vi "电缸控制.vi"(1 "步序号":u32, 2 "枚举":enum16{"开机", "返回原点", "定位运转", "报警复位"}(ring), 3 "输出设备":tag) -> (0 "error out":errorcluster caption="错误输出")   [LabVIEW 2014]
uses:
  <vilib>/DAQmx/create/channels.llb/DAQmx Create Channel (DO-Digital Output).vi
  <vilib>/DAQmx/write.llb/DAQmx Write (Digital 1D Bool 1Chan 1Samp).vi
panel:
  in  "步信息":T1
  in  "人工输出":T2
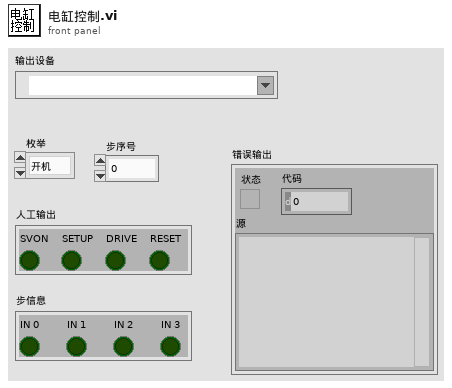
[diagram p1: front panel]
types:
  T1 = cluster{"IN 0":bool, "IN 1":bool, "IN 2":bool, "IN 3":bool}
  T2 = cluster{"SVON":bool, "SETUP":bool, "DRIVE":bool, "RESET":bool}
  T3 = cluster{"Boolean array[0]":bool, "Boolean array[1]":bool, "Boolean array[2]":bool, "Boolean array[3]":bool}
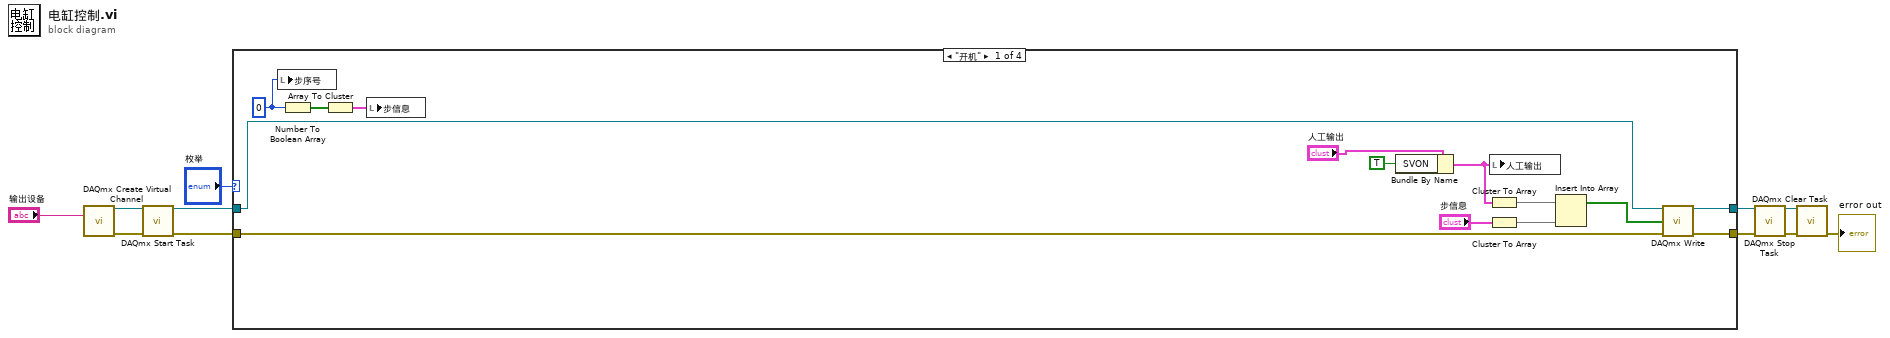
[diagram p0: block diagram]
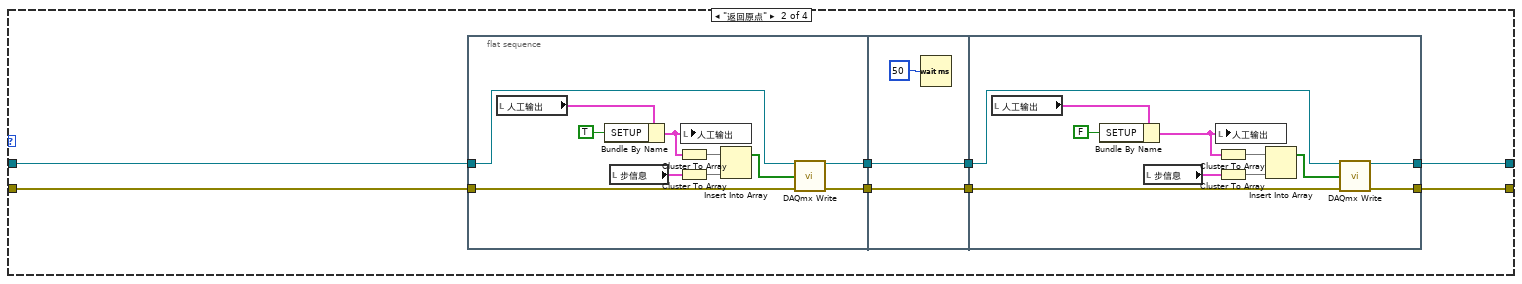
[diagram p2: hidden frame]
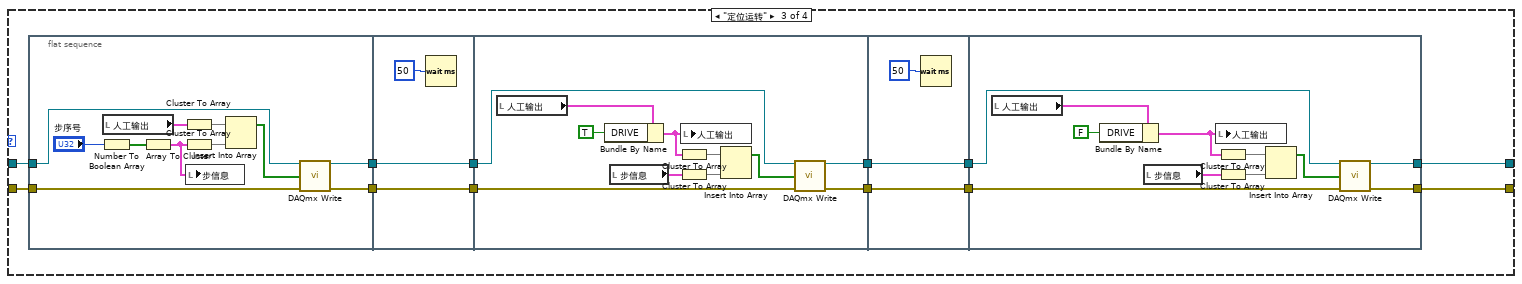
[diagram p3: hidden frame]
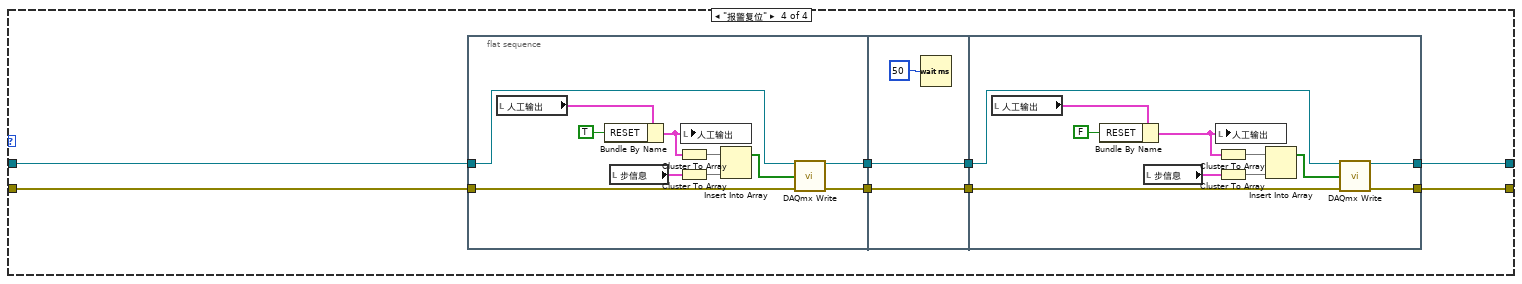
[diagram p4: hidden frame]
diagram:
  n1 = call-poly <vilib>:"DAQmx Create Virtual Channel.vi"("lines"="输出设备") -> ("task out"=w9:refnum<k21>, "error out"=w10:errorcluster)  [unwired: 13 in]
  n2 = call <vilib>:"DAQmx Start Task.vi"("task/channels in"=w9, "error in"=w10) -> ("task out"=w8:refnum<k21>, "error out"=w7:errorcluster)  [unwired: 12 in]
  n3 = case shown="\"开机\"" "枚举" {
    tunnel: w8 -> [w22 w33 w70 w117]
    tunnel: w7 -> [w21 w32 w69 w116]
    tunnel: [w19 w31 w64 w111] -> w3
    tunnel: [w18 w30 w63 w110] -> w2
    frame "开机" {
      w14 = 0
      n4 = local write "步序号"(w14) -> ()
      n5 = Number To Boolean Array(number=w14) -> (Boolean array=w13:bool[])
      n6 = Array To Cluster(array=w13) -> (cluster=w12:T3)
      n7 = local write "步信息"(w12) -> ()
      n8 = Bundle By Name(cluster="人工输出", "SVON"=TRUE) -> (w15:T2)
      n9 = Cluster To Array(cluster=w15) -> (array=w24:bool[])
      n10 = Cluster To Array(cluster="步信息") -> (array=w23:bool[])
      n11 = local write "人工输出"(w15) -> ()
      n12 = Insert Into Array(array=w24, new element=w23) -> (w20:bool[])  [unwired: 1 in]
      n13 = call-poly <vilib>:"DAQmx Write.vi"("task/channels in"=w22, "data"=w20, "error in"=w21) -> ("task out"=w19:refnum<k21>, "error out"=w18:errorcluster)  [unwired: 10 in, 1 out]
    }
    frame "返回原点" {
      n14 = flat-sequence {
        tunnel: w33 -> [w44]
        tunnel: w32 -> [w43]
        tunnel: [w36] -> w29
        tunnel: [w35] -> w27
        tunnel: w29 -> [w46]
        tunnel: [w46] -> w28
        tunnel: w27 -> [w45]
        tunnel: [w45] -> w26
        tunnel: [w58] -> w31
        tunnel: [w57] -> w30
        tunnel: w28 -> [w49]
        tunnel: w26 -> [w48]
        frame #0 {
          n15 = local read "人工输出"() -> (w42:T2)
          n16 = Bundle By Name(cluster=w42, "SETUP"=TRUE) -> (w40:T2)
          n17 = local read "步信息"() -> (w38:T1)
          n18 = Cluster To Array(cluster=w40) -> (array=w39:bool[])
          n19 = Cluster To Array(cluster=w38) -> (array=w34:bool[])
          n20 = local write "人工输出"(w40) -> ()
          n21 = Insert Into Array(array=w39, new element=w34) -> (w37:bool[])  [unwired: 1 in]
          n22 = call-poly <vilib>:"DAQmx Write.vi"("task/channels in"=w44, "data"=w37, "error in"=w43) -> ("task out"=w36:refnum<k21>, "error out"=w35:errorcluster)  [unwired: 10 in, 1 out]
        }
        frame #1 {
          n23 = Wait (ms)(milliseconds to wait=u32 50 ("等待时间（毫秒）")) -> ()  [unwired: 1 out]
        }
        frame #2 {
          n24 = local read "人工输出"() -> (w56:T2)
          n25 = Bundle By Name(cluster=w56, "SETUP"=FALSE) -> (w54:T2)
          n26 = local read "步信息"() -> (w53:T1)
          n27 = local write "人工输出"(w54) -> ()
          n28 = Cluster To Array(cluster=w54) -> (array=w52:bool[])
          n29 = Cluster To Array(cluster=w53) -> (array=w51:bool[])
          n30 = Insert Into Array(array=w52, new element=w51) -> (w50:bool[])  [unwired: 1 in]
          n31 = call-poly <vilib>:"DAQmx Write.vi"("task/channels in"=w49, "data"=w50, "error in"=w48) -> ("task out"=w58:refnum<k21>, "error out"=w57:errorcluster)  [unwired: 10 in, 1 out]
        }
      }
    }
    frame "定位运转" {
      n32 = flat-sequence {
        tunnel: w70 -> [w76]
        tunnel: w69 -> [w75]
        tunnel: [w72] -> w68
        tunnel: [w71] -> w65
        tunnel: w68 -> [w83]
        tunnel: [w83] -> w67
        tunnel: [w82] -> w66
        tunnel: w65 -> [w82]
        tunnel: w67 -> [w95]
        tunnel: w66 -> [w94]
        tunnel: [w86] -> w62
        tunnel: [w85] -> w59
        tunnel: w62 -> [w97]
        tunnel: [w97] -> w61
        tunnel: [w96] -> w60
        tunnel: w59 -> [w96]
        tunnel: [w107] -> w64
        tunnel: [w106] -> w63
        tunnel: w61 -> [w105]
        tunnel: w60 -> [w104]
        frame #0 {
          n33 = Number To Boolean Array(number="步序号") -> (Boolean array=w80:bool[])
          n34 = local read "人工输出"() -> (w78:T2)
          n35 = Array To Cluster(array=w80) -> (cluster=w73:T3)
          n36 = Cluster To Array(cluster=w78) -> (array=w77:bool[])
          n37 = Cluster To Array(cluster=w73) -> (array=w79:bool[])
          n38 = local write "步信息"(w73) -> ()
          n39 = Insert Into Array(array=w77, new element=w79) -> (w74:bool[])  [unwired: 1 in]
          n40 = call-poly <vilib>:"DAQmx Write.vi"("task/channels in"=w76, "data"=w74, "error in"=w75) -> ("task out"=w72:refnum<k21>, "error out"=w71:errorcluster)  [unwired: 10 in, 1 out]
        }
        frame #1 {
          n41 = Wait (ms)(milliseconds to wait=u32 50 ("毫秒倍数")) -> ()  [unwired: 1 out]
        }
        frame #2 {
          n42 = local read "人工输出"() -> (w93:T2)
          n43 = Bundle By Name(cluster=w93, "DRIVE"=TRUE) -> (w91:T2)
          n44 = local read "步信息"() -> (w90:T1)
          n45 = Cluster To Array(cluster=w91) -> (array=w89:bool[])
          n46 = Cluster To Array(cluster=w90) -> (array=w88:bool[])
          n47 = local write "人工输出"(w91) -> ()
          n48 = Insert Into Array(array=w89, new element=w88) -> (w87:bool[])  [unwired: 1 in]
          n49 = call-poly <vilib>:"DAQmx Write.vi"("task/channels in"=w95, "data"=w87, "error in"=w94) -> ("task out"=w86:refnum<k21>, "error out"=w85:errorcluster)  [unwired: 10 in, 1 out]
        }
        frame #3 {
          n50 = Wait (ms)(milliseconds to wait=u32 50 ("毫秒倍数")) -> ()  [unwired: 1 out]
        }
        frame #4 {
          n51 = local read "人工输出"() -> (w109:T2)
          n52 = Bundle By Name(cluster=w109, "DRIVE"=FALSE) -> (w103:T2)
          n53 = local read "步信息"() -> (w102:T1)
          n54 = local write "人工输出"(w103) -> ()
          n55 = Cluster To Array(cluster=w103) -> (array=w101:bool[])
          n56 = Cluster To Array(cluster=w102) -> (array=w100:bool[])
          n57 = Insert Into Array(array=w101, new element=w100) -> (w99:bool[])  [unwired: 1 in]
          n58 = call-poly <vilib>:"DAQmx Write.vi"("task/channels in"=w105, "data"=w99, "error in"=w104) -> ("task out"=w107:refnum<k21>, "error out"=w106:errorcluster)  [unwired: 10 in, 1 out]
        }
      }
    }
    frame "报警复位" {
      n59 = flat-sequence {
        tunnel: w117 -> [w128]
        tunnel: w116 -> [w127]
        tunnel: [w119] -> w115
        tunnel: [w118] -> w112
        tunnel: w115 -> [w130]
        tunnel: [w130] -> w114
        tunnel: [w129] -> w113
        tunnel: w112 -> [w129]
        tunnel: w114 -> [w136]
        tunnel: w113 -> [w135]
        tunnel: [w133] -> w111
        tunnel: [w132] -> w110
        frame #0 {
          n60 = local read "人工输出"() -> (w126:T2)
          n61 = Bundle By Name(cluster=w126, "RESET"=TRUE) -> (w124:T2)
          n62 = local read "步信息"() -> (w123:T1)
          n63 = Cluster To Array(cluster=w124) -> (array=w122:bool[])
          n64 = Cluster To Array(cluster=w123) -> (array=w121:bool[])
          n65 = local write "人工输出"(w124) -> ()
          n66 = Insert Into Array(array=w122, new element=w121) -> (w120:bool[])  [unwired: 1 in]
          n67 = call-poly <vilib>:"DAQmx Write.vi"("task/channels in"=w128, "data"=w120, "error in"=w127) -> ("task out"=w119:refnum<k21>, "error out"=w118:errorcluster)  [unwired: 10 in, 1 out]
        }
        frame #1 {
          n68 = Wait (ms)(milliseconds to wait=u32 50 ("毫秒倍数")) -> ()  [unwired: 1 out]
        }
        frame #2 {
          n69 = local read "人工输出"() -> (w141:T2)
          n70 = Bundle By Name(cluster=w141, "RESET"=FALSE) -> (w137:T2)
          n71 = local read "步信息"() -> (w138:T1)
          n72 = local write "人工输出"(w137) -> ()
          n73 = Cluster To Array(cluster=w137) -> (array=w140:bool[])
          n74 = Cluster To Array(cluster=w138) -> (array=w139:bool[])
          n75 = Insert Into Array(array=w140, new element=w139) -> (w134:bool[])  [unwired: 1 in]
          n76 = call-poly <vilib>:"DAQmx Write.vi"("task/channels in"=w136, "data"=w134, "error in"=w135) -> ("task out"=w133:refnum<k21>, "error out"=w132:errorcluster)  [unwired: 10 in, 1 out]
        }
      }
    }
  }
  n77 = call <vilib>:"DAQmx Stop Task.vi"("task/channels in"=w3, "error in"=w2) -> ("task out"=w6:refnum<k21>, "error out"=w5:errorcluster)  [unwired: 12 in]
  n78 = call <vilib>:"DAQmx Clear Task.vi"("task in"=w6, "error in"=w5) -> ("error out"=→"error out":errorcluster)  [unwired: 13 in]
